vi "SeqEditor_getConPanekids.vi"(11 "steppath":path) -> (2 "OUTPUT":T1[](array[typedef]), 3 "INPUT":T1[](array[typedef]))   [LabVIEW 2017, in "NLTest.lvclass"]
uses:
  NLTest.lvclass
  VISTEP_class_INOUTPUT.ctl
  VISTEP_class_INOUTPUT_TYPE.ctl
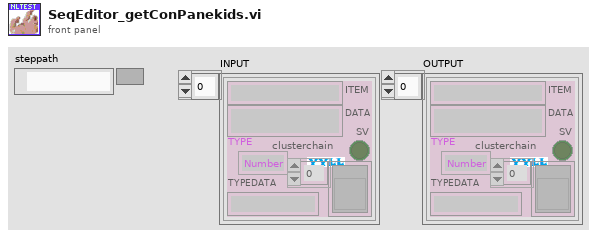
[diagram p1: front panel]
types:
  T1 = typedef "NLTest.lvclass/VISTEP_class_INOUTPUT.ctl" = cluster{"ITEM":string, "DATA":string, "TYPE":T2, "TYPEDATA":string, "SV":bool, "clusterchain":refnum<vi>[]}
  T2 = typedef "NLTest.lvclass/VISTEP_class_INOUTPUT_TYPE.ctl" = enum16{"Number", "String", "Bool", "Enum", "Path", "VISA", "NA"}
  T3 = cluster{"ctl":refnum<vi>, "clusterchain":refnum<vi>[]}[]
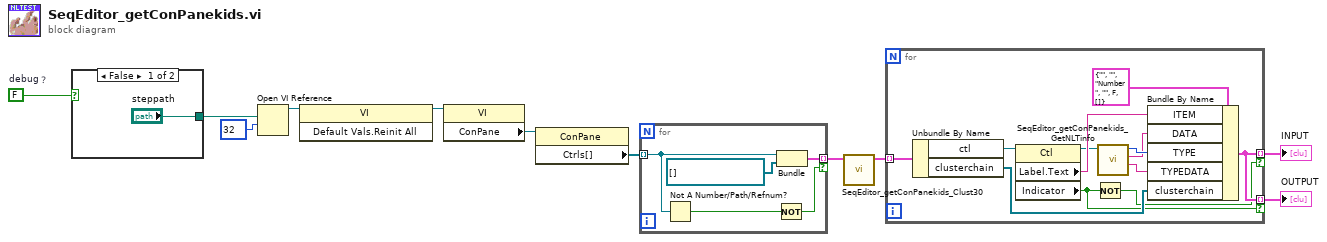
[diagram p0: block diagram]
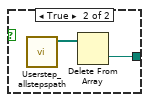
[diagram p2: hidden frame]
diagram:
  w1 = FALSE  # debug？
  n1 = case shown="False" w1 {
    tunnel: ["steppath" w13] -> w2
    frame False {
    }
    frame True {
      n2 = call "Userstep_allstepspath.vi"() -> ("Array"=w14:path[])  [unwired: 11 in]
      n3 = Delete From Array(array=w14) -> (deleted portion=w13:path)  [unwired: 2 in, 1 out]
    }
  }
  n4 = Open VI Reference(vi path=w2, options=32) -> (vi reference=w5:refnum<vi>)  [unwired: 4 in, 1 out]
  n5 = invoke class="VI" method="Default Vals.Reinit All"(reference=w5) -> (reference out=w4:refnum<vi>)  [unwired: 2 in, 2 out]
  n6 = property class="VI"(reference=w4) -> ("ConPane"=w3:refnum<vi>)  [unwired: 1 in, 2 out]
  n7 = property class="ConPane"(reference=w3) -> ("Ctrls[]"=w11:refnum<vi>[])  [unwired: 1 in, 2 out]
  n8 = for {
    tunnel: w11 -> [w16] mode=indexing
    tunnel: [w15] -> w10 mode=indexing if=w18
    n9 = Not A Number/Path/Refnum?(number/path/refnum=w16) -> (NaN/Path/Refnum?=w19:bool)
    n10 = Not(x=w19) -> (.not. x?=w18:bool)
    n11 = Bundle(w16, "clusterchain"=refnum<vi>[] []) -> (w15:cluster{refnum<vi>, "clusterchain":refnum<vi>[]})  [unwired: 1 in]
  }
  n12 = call "SeqEditor_getConPanekids_Clust30.vi"("Array"=w10) -> ("Array 2"=w9:T3)  [unwired: 10 in]
  n13 = for {
    tunnel: w9 -> [w31] mode=indexing
    tunnel: [w26] -> w8 mode=indexing if=w24
    tunnel: [w26] -> w7 mode=indexing if=w25
    n14 = Unbundle By Name(w31) -> ("ctl"=w30:refnum<vi>, "clusterchain"=w28:refnum<vi>[])
    n15 = property class="Ctl"(reference=w30) -> (reference out=w23:refnum<vi>, "Label.Text"=w27:string, "Indicator"=w25:bool)  [unwired: 1 in, 1 out]
    n16 = Not(x=w25) -> (.not. x?=w24:bool)
    n17 = call "SeqEditor_getConPanekids_GetNLTinfo.vi"("reference in"=w23) -> ("typedata"=w20:string, "CtrlTextValue"=w21:string, "TYPE"=w22:T2)  [unwired: 8 in]
    n18 = Bundle By Name(cluster=T1 {"ITEM"="", "DATA"="", "TYPE"=enum."Number", "TYPEDATA"="", "SV"=FALSE, "clusterchain"=[]} ("Cluster"), "ITEM"=w27, "DATA"=w21, "TYPE"=w22, "TYPEDATA"=w20, "clusterchain"=w28) -> (w26:T1)
  }
  "INPUT" <- w8
  "OUTPUT" <- w7
